vi "Error.vi"(8 "error in (no error)":errorcluster, 11 "Name":string) -> (0 "error out":errorcluster)   [LabVIEW 2021, in "Config Library.lvlib" / "json class.lvclass"]
uses:
  json class.lvclass
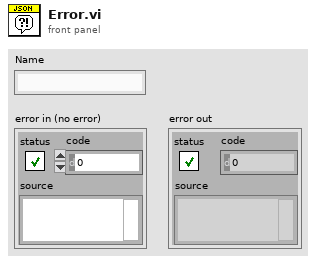
[diagram p1: front panel]
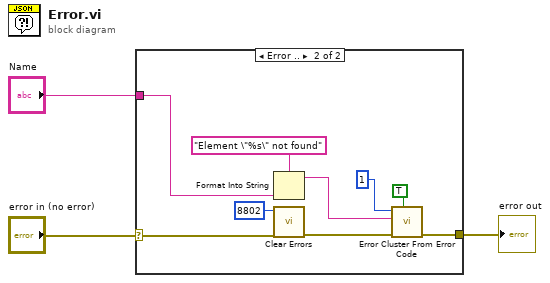
[diagram p0: block diagram]
diagram:
  n1 = case shown="Error .." "error in (no error)" {
    selector: "error in (no error)" -> [w4 w6]
    tunnel: [w4 w13] -> w2
    tunnel: "Name" -> [_ w10]
    frame No Error {
    }
    frame Error {
      n2 = Format Into String(format string="Element \"%s\" not found", w10) -> (resulting string=w11:string)  [unwired: 2 in, 1 out]
      n3 = call <vilib>:"Clear Errors.vi"("error in (no error)"=w6, "specific error code to clear (0: all)"=8802) -> ("error out"=w5:errorcluster)  [unwired: 4 in, 1 out]
      n4 = call <vilib>:"Error Cluster From Error Code.vi"("show call chain? (False)"=TRUE, "error in (no error)"=w5, "error message (\"\")"=w11, "error code (0)"=1) -> ("error out"=w13:errorcluster)  [unwired: 5 in]
    }
  }
  "error out" <- w2
